vi "GetSetBlackLevel.vi"(7 "Set?":bool, 8 "error in (no error)":errorcluster, 10 "Value in":dbl, 11 "Camera in":refnum<class "Camera.lvclass">) -> (0 "error out":errorcluster, 2 "Value out":dbl)   [LabVIEW 2020, in "Camera.lvclass"]
uses:
  Camera.lvclass
  Camera.lvclass/Camera.ctl
  bin/gindustrialcam_32-1.dll
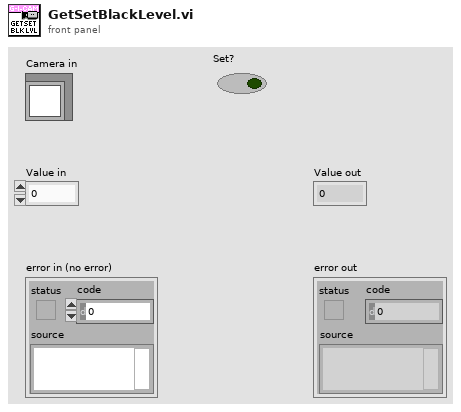
[diagram p1: front panel]
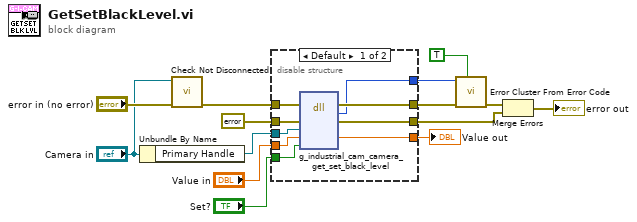
[diagram p0: block diagram]
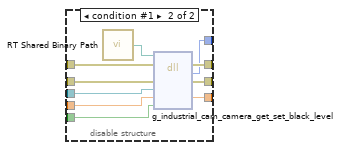
[diagram p2: hidden frame]
diagram:
  n1 = Unbundle By Name("Camera in") -> ("Primary Handle"=w5:refnum<data-value>)
  n2 = call "Check Not Disconnected.vi"("error in (no error)"="error in (no error)", "Camera in"="Camera in") -> ("error out"=w4:errorcluster)  [unwired: 9 in]
  n3 = disable-structure shown="Default" {
    disable-tunnel: [w23 w33] -> w14
    disable-tunnel: [w22 w32] -> w13
    disable-tunnel: [w21 w31] -> w11
    disable-tunnel: errorcluster {"status"=FALSE, "code"=0, "source"=""} ("error constant") -> [w20 w30]
    disable-tunnel: "Set?" -> [w19 w29]
    disable-tunnel: w5 -> [w18 w28]
    disable-tunnel: w4 -> [w17 w27]
    disable-tunnel: "Value in" -> [w16 w26]
    disable-tunnel: [w15 w25] -> w1
    frame condition #0 (active) {
      n4 = dll-call lib="C:/serenial/lib/g-industrial-camera/LabVIEW/g_industrial_cam/bin/gindustrialcam_*-1.*" fn="g_industrial_cam_camera_get_set_black_level"(error in=w17, "err"=w20, "edvr"=w18, "value"=w16, "set"=w19) -> (error out=w23:errorcluster, "Mg_Error"=w22:i32, "err"=w21:errorcluster, "value"=w15:dbl)  [unwired: 4 in, 1 out]
    }
    frame condition #1 {
      n5 = call "RT Shared Binary Path.vi"() -> ("Path"=w24:path)
      n6 = dll-call lib="C:/serenial/lib/g-industrial-camera/LabVIEW/g_industrial_cam/bin/gindustrialcam_*-1.*" fn="g_industrial_cam_camera_get_set_black_level"(path in=w24, error in=w27, "err"=w30, "edvr"=w28, "value"=w26, "set"=w29) -> (error out=w33:errorcluster, "Mg_Error"=w32:i32, "err"=w31:errorcluster, "value"=w25:dbl)  [unwired: 3 in, 1 out]
    }
  }
  "Value out" <- w1
  n7 = call <vilib>:"Error Cluster From Error Code.vi"("show call chain? (False)"=TRUE, "error in (no error)"=w14, "error code (0)"=w13) -> ("error out"=w12:errorcluster)  [unwired: 6 in]
  n8 = Merge Errors(w12, w11) -> (→"error out":errorcluster)
